vi "PicoScope6000aSettings.vi"(0 "handle in":i16=16384, 1 "Device Info":T3={"PICO_DRIVER_VERSION"="", "PICO_USB_VERSION"="", "PICO_HARDWARE_VERSION"="", "PICO_VARIANT_INFO"="", "PICO_BATCH_AND_SERIAL"="", "PICO_CAL_DATE"="", "PICO_KERNEL_VERSION"="", "PICO_DIGITAL_HARDWARE_VERSION"="", "PICO_ANALOGUE_HARDWARE_VERSION"="", "PICO_FIRMWARE_VERSION_1"="", "PICO_FIRMWARE_VERSION_2"="", "PICO_IPP_VERSION"="", "PICO_DRIVER_PATH"="", "PICO_FIRMWARE_VERSION_3"="", "PICO_FRONT_PANEL_FIRMWARE_VERSION"="", "Number of Channels"=0, "MSO"=TRUE}, 2 "Channels":T2={"Channel A Settings "={"Enabled"=FALSE, "Coupling"=50, "Range"=5, "Analogue Offset"=0.0, "BandWidth"=0}, "Channel B Settings "={"Enabled"=FALSE, "Coupling"=50, "Range"=5, "Analogue Offset"=0.0, "BandWidth"=0}, "Channel C Settings "={"Enabled"=FALSE, "Coupling"=50, "Range"=5, "Analogue Offset"=0.0, "BandWidth"=0}, "Channel D Settings "={"Enabled"=FALSE, "Coupling"=50, "Range"=5, "Analogue Offset"=0.0, "BandWidth"=0}, "Channel E Settings "={"Enabled"=FALSE, "Coupling"=50, "Range"=5, "Analogue Offset"=0.0, "BandWidth"=0}, "Channel F Settings "={"Enabled"=FALSE, "Coupling"=50, "Range"=5, "Analogue Offset"=0.0, "BandWidth"=0}, "Channel G Settings "={"Enabled"=FALSE, "Coupling"=50, "Range"=5, "Analogue Offset"=0.0, "BandWidth"=0}, "Channel H Settings "={"Enabled"=FALSE, "Coupling"=50, "Range"=5, "Analogue Offset"=0.0, "BandWidth"=0}} {"Channel H Settings"."BandWidth" items=["Full"=0, "100kHz"=100000, "20kHz"=200000, "1MHz"=1000000, "20MHz"=20000000, "25MHz"=25000000, "50MHz"=50000000, "200MHz"=200000000, "250MHz"=250000000, "500MHz"=500000000]; "Channel H Settings"."Range" items=["10mV"=0, "20mV"=1, "50mV"=2, "100mV"=3, "200mV"=4, "500mV"=5, "1V"=6, "2V"=7, "5V"=8, "10V"=9, "20V"=10, "50V"=11, "100V"=12, "200V"=13, "x10_Probe_100mV"=32, "x10_Probe_200mV"=33, "x10_Probe_500mV"=34, "x10_Probe_1V"=35, "x10_Probe_2V"=36, "x10_Probe_5V"=37, "x10_Probe_10V"=38, "x10_Probe_20V"=39, "x10_Probe_50V"=40, "x10_Probe_100V"=41, "x10_Probe_200V"=42, "x10_Probe_500V"=43, "CURRENT_CLAMP_60A_2A"=10500, "CURRENT_CLAMP_60A_5A"=10501, "CURRENT_CLAMP_60A_10A"=10502, "CURRENT_CLAMP_60A_20A"=10503, "CURRENT_CLAMP_60A_50A"=10504, "CURRENT_CLAMP_60A_60A"=10505, "CURRENT_CLAMP_60A_V2_0_5A"=10600, "CURRENT_CLAMP_60A_V2_1A"=10601, "CURRENT_CLAMP_60A_V2_2A"=10602, "CURRENT_CLAMP_60A_V2_5A"=10603, "CURRENT_CLAMP_60A_V2_10A"=10604, "CURRENT_CLAMP_60A_V2_20A"=10605, "CURRENT_CLAMP_60A_V2_50A"=10606, "CURRENT_CLAMP_60A_V2_60A"=10607, "RESISTANCE_LEAD_NEG5_TO_20OHM"=7000, "RESISTANCE_LEAD_NEG50_TO_200OHM"=7001, "RESISTANCE_LEAD_NEG500_TO_2KOHM"=7002, "RESISTANCE_LEAD_NEG5K_TO_20KOHM"=7003, "RESISTANCE_LEAD_NEG50K_TO_LEAD_200KOHM"=7004, "RESISTANCE_LEAD_NEG500K_TO_LEAD_2MOHM"=7005, "RESISTANCE_LEAD_DIODE_TEST"=7006, "HT_NEG3_TO_5KV"=8950, "HT_NEG3_TO_10KV"=8951, "HT_NEG5_TO_20KV"=8952, "HT_NEG5_TO_50KV"=8953, "HT_NEG5_TO_100KV"=8954, "HT_NEG3_TO_5KV_INVERTED"=8955, "HT_NEG3_TO_10KV_INVERTED"=8956, "HT_NEG5_TO_20KV_INVERTED"=8957, "HT_NEG5_TO_50KV_INVERTED"=8958, "HT_NEG5_TO_100KV_INVERTED"=8959, "TEMPERATURE_NEG50_TO_150DEGC"=9000, "PRESSURE_SENSOR_-100k-150k_PASCALS"=9100, "PRESSURE_SENSOR_-100k_TO_400k_PASCALS"=9101, "PRESSURE_SENSOR_-200k_TO_800k_PASCALS"=9102, "PRESSURE_SENSOR_-400k_TO_1600k_PASCALS"=9103, "PRESSURE_SENSOR_-400k_TO_3400k_PASCALS"=9104, "PRESSURE_SENSOR_-150k_TO_1350k_PASCALS"=9105]; "Channel H Settings"."Coupling" items=["AC"=0, "DC 1M Ohm"=1, "DC 50 Ohm"=50]; "Channel G Settings"."BandWidth" items=["Full"=0, "100kHz"=100000, "20kHz"=200000, "1MHz"=1000000, "20MHz"=20000000, "25MHz"=25000000, "50MHz"=50000000, "200MHz"=200000000, "250MHz"=250000000, "500MHz"=500000000]; "Channel G Settings"."Range" items=["10mV"=0, "20mV"=1, "50mV"=2, "100mV"=3, "200mV"=4, "500mV"=5, "1V"=6, "2V"=7, "5V"=8, "10V"=9, "20V"=10, "50V"=11, "100V"=12, "200V"=13, "x10_Probe_100mV"=32, "x10_Probe_200mV"=33, "x10_Probe_500mV"=34, "x10_Probe_1V"=35, "x10_Probe_2V"=36, "x10_Probe_5V"=37, "x10_Probe_10V"=38, "x10_Probe_20V"=39, "x10_Probe_50V"=40, "x10_Probe_100V"=41, "x10_Probe_200V"=42, "x10_Probe_500V"=43, "CURRENT_CLAMP_60A_2A"=10500, "CURRENT_CLAMP_60A_5A"=10501, "CURRENT_CLAMP_60A_10A"=10502, "CURRENT_CLAMP_60A_20A"=10503, "CURRENT_CLAMP_60A_50A"=10504, "CURRENT_CLAMP_60A_60A"=10505, "CURRENT_CLAMP_60A_V2_0_5A"=10600, "CURRENT_CLAMP_60A_V2_1A"=10601, "CURRENT_CLAMP_60A_V2_2A"=10602, "CURRENT_CLAMP_60A_V2_5A"=10603, "CURRENT_CLAMP_60A_V2_10A"=10604, "CURRENT_CLAMP_60A_V2_20A"=10605, "CURRENT_CLAMP_60A_V2_50A"=10606, "CURRENT_CLAMP_60A_V2_60A"=10607, "RESISTANCE_LEAD_NEG5_TO_20OHM"=7000, "RESISTANCE_LEAD_NEG50_TO_200OHM"=7001, "RESISTANCE_LEAD_NEG500_TO_2KOHM"=7002, "RESISTANCE_LEAD_NEG5K_TO_20KOHM"=7003, "RESISTANCE_LEAD_NEG50K_TO_LEAD_200KOHM"=7004, "RESISTANCE_LEAD_NEG500K_TO_LEAD_2MOHM"=7005, "RESISTANCE_LEAD_DIODE_TEST"=7006, "HT_NEG3_TO_5KV"=8950, "HT_NEG3_TO_10KV"=8951, "HT_NEG5_TO_20KV"=8952, "HT_NEG5_TO_50KV"=8953, "HT_NEG5_TO_100KV"=8954, "HT_NEG3_TO_5KV_INVERTED"=8955, "HT_NEG3_TO_10KV_INVERTED"=8956, "HT_NEG5_TO_20KV_INVERTED"=8957, "HT_NEG5_TO_50KV_INVERTED"=8958, "HT_NEG5_TO_100KV_INVERTED"=8959, "TEMPERATURE_NEG50_TO_150DEGC"=9000, "PRESSURE_SENSOR_-100k-150k_PASCALS"=9100, "PRESSURE_SENSOR_-100k_TO_400k_PASCALS"=9101, "PRESSURE_SENSOR_-200k_TO_800k_PASCALS"=9102, "PRESSURE_SENSOR_-400k_TO_1600k_PASCALS"=9103, "PRESSURE_SENSOR_-400k_TO_3400k_PASCALS"=9104, "PRESSURE_SENSOR_-150k_TO_1350k_PASCALS"=9105]; "Channel G Settings"."Coupling" items=["AC"=0, "DC 1M Ohm"=1, "DC 50 Ohm"=50]; "Channel F Settings"."BandWidth" items=["Full"=0, "100kHz"=100000, "20kHz"=200000, "1MHz"=1000000, "20MHz"=20000000, "25MHz"=25000000, "50MHz"=50000000, "200MHz"=200000000, "250MHz"=250000000, "500MHz"=500000000]; "Channel F Settings"."Range" items=["10mV"=0, "20mV"=1, "50mV"=2, "100mV"=3, "200mV"=4, "500mV"=5, "1V"=6, "2V"=7, "5V"=8, "10V"=9, "20V"=10, "50V"=11, "100V"=12, "200V"=13, "x10_Probe_100mV"=32, "x10_Probe_200mV"=33, "x10_Probe_500mV"=34, "x10_Probe_1V"=35, "x10_Probe_2V"=36, "x10_Probe_5V"=37, "x10_Probe_10V"=38, "x10_Probe_20V"=39, "x10_Probe_50V"=40, "x10_Probe_100V"=41, "x10_Probe_200V"=42, "x10_Probe_500V"=43, "CURRENT_CLAMP_60A_2A"=10500, "CURRENT_CLAMP_60A_5A"=10501, "CURRENT_CLAMP_60A_10A"=10502, "CURRENT_CLAMP_60A_20A"=10503, "CURRENT_CLAMP_60A_50A"=10504, "CURRENT_CLAMP_60A_60A"=10505, "CURRENT_CLAMP_60A_V2_0_5A"=10600, "CURRENT_CLAMP_60A_V2_1A"=10601, "CURRENT_CLAMP_60A_V2_2A"=10602, "CURRENT_CLAMP_60A_V2_5A"=10603, "CURRENT_CLAMP_60A_V2_10A"=10604, "CURRENT_CLAMP_60A_V2_20A"=10605, "CURRENT_CLAMP_60A_V2_50A"=10606, "CURRENT_CLAMP_60A_V2_60A"=10607, "RESISTANCE_LEAD_NEG5_TO_20OHM"=7000, "RESISTANCE_LEAD_NEG50_TO_200OHM"=7001, "RESISTANCE_LEAD_NEG500_TO_2KOHM"=7002, "RESISTANCE_LEAD_NEG5K_TO_20KOHM"=7003, "RESISTANCE_LEAD_NEG50K_TO_LEAD_200KOHM"=7004, "RESISTANCE_LEAD_NEG500K_TO_LEAD_2MOHM"=7005, "RESISTANCE_LEAD_DIODE_TEST"=7006, "HT_NEG3_TO_5KV"=8950, "HT_NEG3_TO_10KV"=8951, "HT_NEG5_TO_20KV"=8952, "HT_NEG5_TO_50KV"=8953, "HT_NEG5_TO_100KV"=8954, "HT_NEG3_TO_5KV_INVERTED"=8955, "HT_NEG3_TO_10KV_INVERTED"=8956, "HT_NEG5_TO_20KV_INVERTED"=8957, "HT_NEG5_TO_50KV_INVERTED"=8958, "HT_NEG5_TO_100KV_INVERTED"=8959, "TEMPERATURE_NEG50_TO_150DEGC"=9000, "PRESSURE_SENSOR_-100k-150k_PASCALS"=9100, "PRESSURE_SENSOR_-100k_TO_400k_PASCALS"=9101, "PRESSURE_SENSOR_-200k_TO_800k_PASCALS"=9102, "PRESSURE_SENSOR_-400k_TO_1600k_PASCALS"=9103, "PRESSURE_SENSOR_-400k_TO_3400k_PASCALS"=9104, "PRESSURE_SENSOR_-150k_TO_1350k_PASCALS"=9105]; "Channel F Settings"."Coupling" items=["AC"=0, "DC 1M Ohm"=1, "DC 50 Ohm"=50]; "Channel E Settings"."BandWidth" items=["Full"=0, "100kHz"=100000, "20kHz"=200000, "1MHz"=1000000, "20MHz"=20000000, "25MHz"=25000000, "50MHz"=50000000, "200MHz"=200000000, "250MHz"=250000000, "500MHz"=500000000]; "Channel E Settings"."Range" items=["10mV"=0, "20mV"=1, "50mV"=2, "100mV"=3, "200mV"=4, "500mV"=5, "1V"=6, "2V"=7, "5V"=8, "10V"=9, "20V"=10, "50V"=11, "100V"=12, "200V"=13, "x10_Probe_100mV"=32, "x10_Probe_200mV"=33, "x10_Probe_500mV"=34, "x10_Probe_1V"=35, "x10_Probe_2V"=36, "x10_Probe_5V"=37, "x10_Probe_10V"=38, "x10_Probe_20V"=39, "x10_Probe_50V"=40, "x10_Probe_100V"=41, "x10_Probe_200V"=42, "x10_Probe_500V"=43, "CURRENT_CLAMP_60A_2A"=10500, "CURRENT_CLAMP_60A_5A"=10501, "CURRENT_CLAMP_60A_10A"=10502, "CURRENT_CLAMP_60A_20A"=10503, "CURRENT_CLAMP_60A_50A"=10504, "CURRENT_CLAMP_60A_60A"=10505, "CURRENT_CLAMP_60A_V2_0_5A"=10600, "CURRENT_CLAMP_60A_V2_1A"=10601, "CURRENT_CLAMP_60A_V2_2A"=10602, "CURRENT_CLAMP_60A_V2_5A"=10603, "CURRENT_CLAMP_60A_V2_10A"=10604, "CURRENT_CLAMP_60A_V2_20A"=10605, "CURRENT_CLAMP_60A_V2_50A"=10606, "CURRENT_CLAMP_60A_V2_60A"=10607, "RESISTANCE_LEAD_NEG5_TO_20OHM"=7000, "RESISTANCE_LEAD_NEG50_TO_200OHM"=7001, "RESISTANCE_LEAD_NEG500_TO_2KOHM"=7002, "RESISTANCE_LEAD_NEG5K_TO_20KOHM"=7003, "RESISTANCE_LEAD_NEG50K_TO_LEAD_200KOHM"=7004, "RESISTANCE_LEAD_NEG500K_TO_LEAD_2MOHM"=7005, "RESISTANCE_LEAD_DIODE_TEST"=7006, "HT_NEG3_TO_5KV"=8950, "HT_NEG3_TO_10KV"=8951, "HT_NEG5_TO_20KV"=8952, "HT_NEG5_TO_50KV"=8953, "HT_NEG5_TO_100KV"=8954, "HT_NEG3_TO_5KV_INVERTED"=8955, "HT_NEG3_TO_10KV_INVERTED"=8956, "HT_NEG5_TO_20KV_INVERTED"=8957, "HT_NEG5_TO_50KV_INVERTED"=8958, "HT_NEG5_TO_100KV_INVERTED"=8959, "TEMPERATURE_NEG50_TO_150DEGC"=9000, "PRESSURE_SENSOR_-100k-150k_PASCALS"=9100, "PRESSURE_SENSOR_-100k_TO_400k_PASCALS"=9101, "PRESSURE_SENSOR_-200k_TO_800k_PASCALS"=9102, "PRESSURE_SENSOR_-400k_TO_1600k_PASCALS"=9103, "PRESSURE_SENSOR_-400k_TO_3400k_PASCALS"=9104, "PRESSURE_SENSOR_-150k_TO_1350k_PASCALS"=9105]; "Channel E Settings"."Coupling" items=["AC"=0, "DC 1M Ohm"=1, "DC 50 Ohm"=50]; "Channel D Settings"."BandWidth" items=["Full"=0, "100kHz"=100000, "20kHz"=200000, "1MHz"=1000000, "20MHz"=20000000, "25MHz"=25000000, "50MHz"=50000000, "200MHz"=200000000, "250MHz"=250000000, "500MHz"=500000000]; "Channel D Settings"."Range" items=["10mV"=0, "20mV"=1, "50mV"=2, "100mV"=3, "200mV"=4, "500mV"=5, "1V"=6, "2V"=7, "5V"=8, "10V"=9, "20V"=10, "50V"=11, "100V"=12, "200V"=13, "x10_Probe_100mV"=32, "x10_Probe_200mV"=33, "x10_Probe_500mV"=34, "x10_Probe_1V"=35, "x10_Probe_2V"=36, "x10_Probe_5V"=37, "x10_Probe_10V"=38, "x10_Probe_20V"=39, "x10_Probe_50V"=40, "x10_Probe_100V"=41, "x10_Probe_200V"=42, "x10_Probe_500V"=43, "CURRENT_CLAMP_60A_2A"=10500, "CURRENT_CLAMP_60A_5A"=10501, "CURRENT_CLAMP_60A_10A"=10502, "CURRENT_CLAMP_60A_20A"=10503, "CURRENT_CLAMP_60A_50A"=10504, "CURRENT_CLAMP_60A_60A"=10505, "CURRENT_CLAMP_60A_V2_0_5A"=10600, "CURRENT_CLAMP_60A_V2_1A"=10601, "CURRENT_CLAMP_60A_V2_2A"=10602, "CURRENT_CLAMP_60A_V2_5A"=10603, "CURRENT_CLAMP_60A_V2_10A"=10604, "CURRENT_CLAMP_60A_V2_20A"=10605, "CURRENT_CLAMP_60A_V2_50A"=10606, "CURRENT_CLAMP_60A_V2_60A"=10607, "RESISTANCE_LEAD_NEG5_TO_20OHM"=7000, "RESISTANCE_LEAD_NEG50_TO_200OHM"=7001, "RESISTANCE_LEAD_NEG500_TO_2KOHM"=7002, "RESISTANCE_LEAD_NEG5K_TO_20KOHM"=7003, "RESISTANCE_LEAD_NEG50K_TO_LEAD_200KOHM"=7004, "RESISTANCE_LEAD_NEG500K_TO_LEAD_2MOHM"=7005, "RESISTANCE_LEAD_DIODE_TEST"=7006, "HT_NEG3_TO_5KV"=8950, "HT_NEG3_TO_10KV"=8951, "HT_NEG5_TO_20KV"=8952, "HT_NEG5_TO_50KV"=8953, "HT_NEG5_TO_100KV"=8954, "HT_NEG3_TO_5KV_INVERTED"=8955, "HT_NEG3_TO_10KV_INVERTED"=8956, "HT_NEG5_TO_20KV_INVERTED"=8957, "HT_NEG5_TO_50KV_INVERTED"=8958, "HT_NEG5_TO_100KV_INVERTED"=8959, "TEMPERATURE_NEG50_TO_150DEGC"=9000, "PRESSURE_SENSOR_-100k-150k_PASCALS"=9100, "PRESSURE_SENSOR_-100k_TO_400k_PASCALS"=9101, "PRESSURE_SENSOR_-200k_TO_800k_PASCALS"=9102, "PRESSURE_SENSOR_-400k_TO_1600k_PASCALS"=9103, "PRESSURE_SENSOR_-400k_TO_3400k_PASCALS"=9104, "PRESSURE_SENSOR_-150k_TO_1350k_PASCALS"=9105]; "Channel D Settings"."Coupling" items=["AC"=0, "DC 1M Ohm"=1, "DC 50 Ohm"=50]; "Channel C Settings"."BandWidth" items=["Full"=0, "100kHz"=100000, "20kHz"=200000, "1MHz"=1000000, "20MHz"=20000000, "25MHz"=25000000, "50MHz"=50000000, "200MHz"=200000000, "250MHz"=250000000, "500MHz"=500000000]; "Channel C Settings"."Range" items=["10mV"=0, "20mV"=1, "50mV"=2, "100mV"=3, "200mV"=4, "500mV"=5, "1V"=6, "2V"=7, "5V"=8, "10V"=9, "20V"=10, "50V"=11, "100V"=12, "200V"=13, "x10_Probe_100mV"=32, "x10_Probe_200mV"=33, "x10_Probe_500mV"=34, "x10_Probe_1V"=35, "x10_Probe_2V"=36, "x10_Probe_5V"=37, "x10_Probe_10V"=38, "x10_Probe_20V"=39, "x10_Probe_50V"=40, "x10_Probe_100V"=41, "x10_Probe_200V"=42, "x10_Probe_500V"=43, "CURRENT_CLAMP_60A_2A"=10500, "CURRENT_CLAMP_60A_5A"=10501, "CURRENT_CLAMP_60A_10A"=10502, "CURRENT_CLAMP_60A_20A"=10503, "CURRENT_CLAMP_60A_50A"=10504, "CURRENT_CLAMP_60A_60A"=10505, "CURRENT_CLAMP_60A_V2_0_5A"=10600, "CURRENT_CLAMP_60A_V2_1A"=10601, "CURRENT_CLAMP_60A_V2_2A"=10602, "CURRENT_CLAMP_60A_V2_5A"=10603, "CURRENT_CLAMP_60A_V2_10A"=10604, "CURRENT_CLAMP_60A_V2_20A"=10605, "CURRENT_CLAMP_60A_V2_50A"=10606, "CURRENT_CLAMP_60A_V2_60A"=10607, "RESISTANCE_LEAD_NEG5_TO_20OHM"=7000, "RESISTANCE_LEAD_NEG50_TO_200OHM"=7001, "RESISTANCE_LEAD_NEG500_TO_2KOHM"=7002, "RESISTANCE_LEAD_NEG5K_TO_20KOHM"=7003, "RESISTANCE_LEAD_NEG50K_TO_LEAD_200KOHM"=7004, "RESISTANCE_LEAD_NEG500K_TO_LEAD_2MOHM"=7005, "RESISTANCE_LEAD_DIODE_TEST"=7006, "HT_NEG3_TO_5KV"=8950, "HT_NEG3_TO_10KV"=8951, "HT_NEG5_TO_20KV"=8952, "HT_NEG5_TO_50KV"=8953, "HT_NEG5_TO_100KV"=8954, "HT_NEG3_TO_5KV_INVERTED"=8955, "HT_NEG3_TO_10KV_INVERTED"=8956, "HT_NEG5_TO_20KV_INVERTED"=8957, "HT_NEG5_TO_50KV_INVERTED"=8958, "HT_NEG5_TO_100KV_INVERTED"=8959, "TEMPERATURE_NEG50_TO_150DEGC"=9000, "PRESSURE_SENSOR_-100k-150k_PASCALS"=9100, "PRESSURE_SENSOR_-100k_TO_400k_PASCALS"=9101, "PRESSURE_SENSOR_-200k_TO_800k_PASCALS"=9102, "PRESSURE_SENSOR_-400k_TO_1600k_PASCALS"=9103, "PRESSURE_SENSOR_-400k_TO_3400k_PASCALS"=9104, "PRESSURE_SENSOR_-150k_TO_1350k_PASCALS"=9105]; "Channel C Settings"."Coupling" items=["AC"=0, "DC 1M Ohm"=1, "DC 50 Ohm"=50]; "Channel B Settings"."BandWidth" items=["Full"=0, "100kHz"=100000, "20kHz"=200000, "1MHz"=1000000, "20MHz"=20000000, "25MHz"=25000000, "50MHz"=50000000, "200MHz"=200000000, "250MHz"=250000000, "500MHz"=500000000]; "Channel B Settings"."Range" items=["10mV"=0, "20mV"=1, "50mV"=2, "100mV"=3, "200mV"=4, "500mV"=5, "1V"=6, "2V"=7, "5V"=8, "10V"=9, "20V"=10, "50V"=11, "100V"=12, "200V"=13, "x10_Probe_100mV"=32, "x10_Probe_200mV"=33, "x10_Probe_500mV"=34, "x10_Probe_1V"=35, "x10_Probe_2V"=36, "x10_Probe_5V"=37, "x10_Probe_10V"=38, "x10_Probe_20V"=39, "x10_Probe_50V"=40, "x10_Probe_100V"=41, "x10_Probe_200V"=42, "x10_Probe_500V"=43, "CURRENT_CLAMP_60A_2A"=10500, "CURRENT_CLAMP_60A_5A"=10501, "CURRENT_CLAMP_60A_10A"=10502, "CURRENT_CLAMP_60A_20A"=10503, "CURRENT_CLAMP_60A_50A"=10504, "CURRENT_CLAMP_60A_60A"=10505, "CURRENT_CLAMP_60A_V2_0_5A"=10600, "CURRENT_CLAMP_60A_V2_1A"=10601, "CURRENT_CLAMP_60A_V2_2A"=10602, "CURRENT_CLAMP_60A_V2_5A"=10603, "CURRENT_CLAMP_60A_V2_10A"=10604, "CURRENT_CLAMP_60A_V2_20A"=10605, "CURRENT_CLAMP_60A_V2_50A"=10606, "CURRENT_CLAMP_60A_V2_60A"=10607, "RESISTANCE_LEAD_NEG5_TO_20OHM"=7000, "RESISTANCE_LEAD_NEG50_TO_200OHM"=7001, "RESISTANCE_LEAD_NEG500_TO_2KOHM"=7002, "RESISTANCE_LEAD_NEG5K_TO_20KOHM"=7003, "RESISTANCE_LEAD_NEG50K_TO_LEAD_200KOHM"=7004, "RESISTANCE_LEAD_NEG500K_TO_LEAD_2MOHM"=7005, "RESISTANCE_LEAD_DIODE_TEST"=7006, "HT_NEG3_TO_5KV"=8950, "HT_NEG3_TO_10KV"=8951, "HT_NEG5_TO_20KV"=8952, "HT_NEG5_TO_50KV"=8953, "HT_NEG5_TO_100KV"=8954, "HT_NEG3_TO_5KV_INVERTED"=8955, "HT_NEG3_TO_10KV_INVERTED"=8956, "HT_NEG5_TO_20KV_INVERTED"=8957, "HT_NEG5_TO_50KV_INVERTED"=8958, "HT_NEG5_TO_100KV_INVERTED"=8959, "TEMPERATURE_NEG50_TO_150DEGC"=9000, "PRESSURE_SENSOR_-100k-150k_PASCALS"=9100, "PRESSURE_SENSOR_-100k_TO_400k_PASCALS"=9101, "PRESSURE_SENSOR_-200k_TO_800k_PASCALS"=9102, "PRESSURE_SENSOR_-400k_TO_1600k_PASCALS"=9103, "PRESSURE_SENSOR_-400k_TO_3400k_PASCALS"=9104, "PRESSURE_SENSOR_-150k_TO_1350k_PASCALS"=9105]; "Channel B Settings"."Coupling" items=["AC"=0, "DC 1M Ohm"=1, "DC 50 Ohm"=50]; "Channel A Settings"."Range" items=["10mV"=0, "20mV"=1, "50mV"=2, "100mV"=3, "200mV"=4, "500mV"=5, "1V"=6, "2V"=7, "5V"=8, "10V"=9, "20V"=10, "50V"=11, "100V"=12, "200V"=13, "x10_Probe_100mV"=32, "x10_Probe_200mV"=33, "x10_Probe_500mV"=34, "x10_Probe_1V"=35, "x10_Probe_2V"=36, "x10_Probe_5V"=37, "x10_Probe_10V"=38, "x10_Probe_20V"=39, "x10_Probe_50V"=40, "x10_Probe_100V"=41, "x10_Probe_200V"=42, "x10_Probe_500V"=43, "CURRENT_CLAMP_60A_2A"=10500, "CURRENT_CLAMP_60A_5A"=10501, "CURRENT_CLAMP_60A_10A"=10502, "CURRENT_CLAMP_60A_20A"=10503, "CURRENT_CLAMP_60A_50A"=10504, "CURRENT_CLAMP_60A_60A"=10505, "CURRENT_CLAMP_60A_V2_0_5A"=10600, "CURRENT_CLAMP_60A_V2_1A"=10601, "CURRENT_CLAMP_60A_V2_2A"=10602, "CURRENT_CLAMP_60A_V2_5A"=10603, "CURRENT_CLAMP_60A_V2_10A"=10604, "CURRENT_CLAMP_60A_V2_20A"=10605, "CURRENT_CLAMP_60A_V2_50A"=10606, "CURRENT_CLAMP_60A_V2_60A"=10607, "RESISTANCE_LEAD_NEG5_TO_20OHM"=7000, "RESISTANCE_LEAD_NEG50_TO_200OHM"=7001, "RESISTANCE_LEAD_NEG500_TO_2KOHM"=7002, "RESISTANCE_LEAD_NEG5K_TO_20KOHM"=7003, "RESISTANCE_LEAD_NEG50K_TO_LEAD_200KOHM"=7004, "RESISTANCE_LEAD_NEG500K_TO_LEAD_2MOHM"=7005, "RESISTANCE_LEAD_DIODE_TEST"=7006, "HT_NEG3_TO_5KV"=8950, "HT_NEG3_TO_10KV"=8951, "HT_NEG5_TO_20KV"=8952, "HT_NEG5_TO_50KV"=8953, "HT_NEG5_TO_100KV"=8954, "HT_NEG3_TO_5KV_INVERTED"=8955, "HT_NEG3_TO_10KV_INVERTED"=8956, "HT_NEG5_TO_20KV_INVERTED"=8957, "HT_NEG5_TO_50KV_INVERTED"=8958, "HT_NEG5_TO_100KV_INVERTED"=8959, "TEMPERATURE_NEG50_TO_150DEGC"=9000, "PRESSURE_SENSOR_-100k-150k_PASCALS"=9100, "PRESSURE_SENSOR_-100k_TO_400k_PASCALS"=9101, "PRESSURE_SENSOR_-200k_TO_800k_PASCALS"=9102, "PRESSURE_SENSOR_-400k_TO_1600k_PASCALS"=9103, "PRESSURE_SENSOR_-400k_TO_3400k_PASCALS"=9104, "PRESSURE_SENSOR_-150k_TO_1350k_PASCALS"=9105]; "Channel A Settings"."BandWidth" items=["Full"=0, "100kHz"=100000, "20kHz"=200000, "1MHz"=1000000, "20MHz"=20000000, "25MHz"=25000000, "50MHz"=50000000, "200MHz"=200000000, "250MHz"=250000000, "500MHz"=500000000]; "Channel A Settings"."Coupling" items=["AC"=0, "DC 1M Ohm"=1, "DC 50 Ohm"=50]}, 7 "Max ADC value":i16=32512, 11 "error in (no error)":errorcluster, 12 "Trigger Settings":T4={"Trigger Enabled"=FALSE, "Trigger Threshold (Volts/Probe Units)"=0.0, "Trigger Direction"=2, "Trigger Delay (samples)"=0, "Auto Trigger Time (us)"=1000000, "Trigger Source"=0} {"Trigger Source" items=["Channel A"=0, "Channel B"=1, "Channel C"=2, "Channel D"=3, "Channel E"=4, "Channel F"=5, "Channel G"=6, "Channel H"=7, "Trigger AUX"=1001]; "Trigger Direction" items=["Above", "Below", "Rising", "Falling", "Rising or Falling"]; "Trigger Threshold (Volts/Probe Units)" format="%#_6p"}, 14 "Digital Channels":T1={"Port 0 Settings "={"Enabled"=FALSE, "Hysteresis"=3, "Threshold Level (Volts)"=[1.0, 1.0, 1.0, 1.0, 1.0, 1.0, 1.0, 1.0]}, "Port 1 Settings"={"Enabled"=FALSE, "Hysteresis"=3, "Threshold Level (Volts)"=[1.0, 1.0, 1.0, 1.0, 1.0, 1.0, 1.0, 1.0]}} {"Port 1 Settings"."Threshold Level (Volts)" format="%#_4p"; "Port 1 Settings"."Hysteresis" items=["PICO_VERY_HIGH_400MV", "PICO_HIGH_200MV", "PICO_NORMAL_100MV", "PICO_LOW_50MV"]; "Port 0 Settings"."Threshold Level (Volts)" format="%#_4p"; "Port 0 Settings"."Hysteresis" items=["PICO_VERY_HIGH_400MV", "PICO_HIGH_200MV", "PICO_NORMAL_100MV", "PICO_LOW_50MV"]}) -> (3 "Enabled array":i16[](array[numeric])=[1, 0, 0, 0, 0, 0, 0, 0, 0, 0], 4 "handle out":i16=16384, 15 "error out":errorcluster)   [LabVIEW 2010]
doc: "Sets up channels and calls setSimpleTrigger"
uses:
  ps6000a.dll
  PicoScope6000aAnalogChannelSettings.ctl
  PicoScope6000aDigitalChannelSettings.ctl
panel:
  # "D8-D15"
  # "DO-D7"
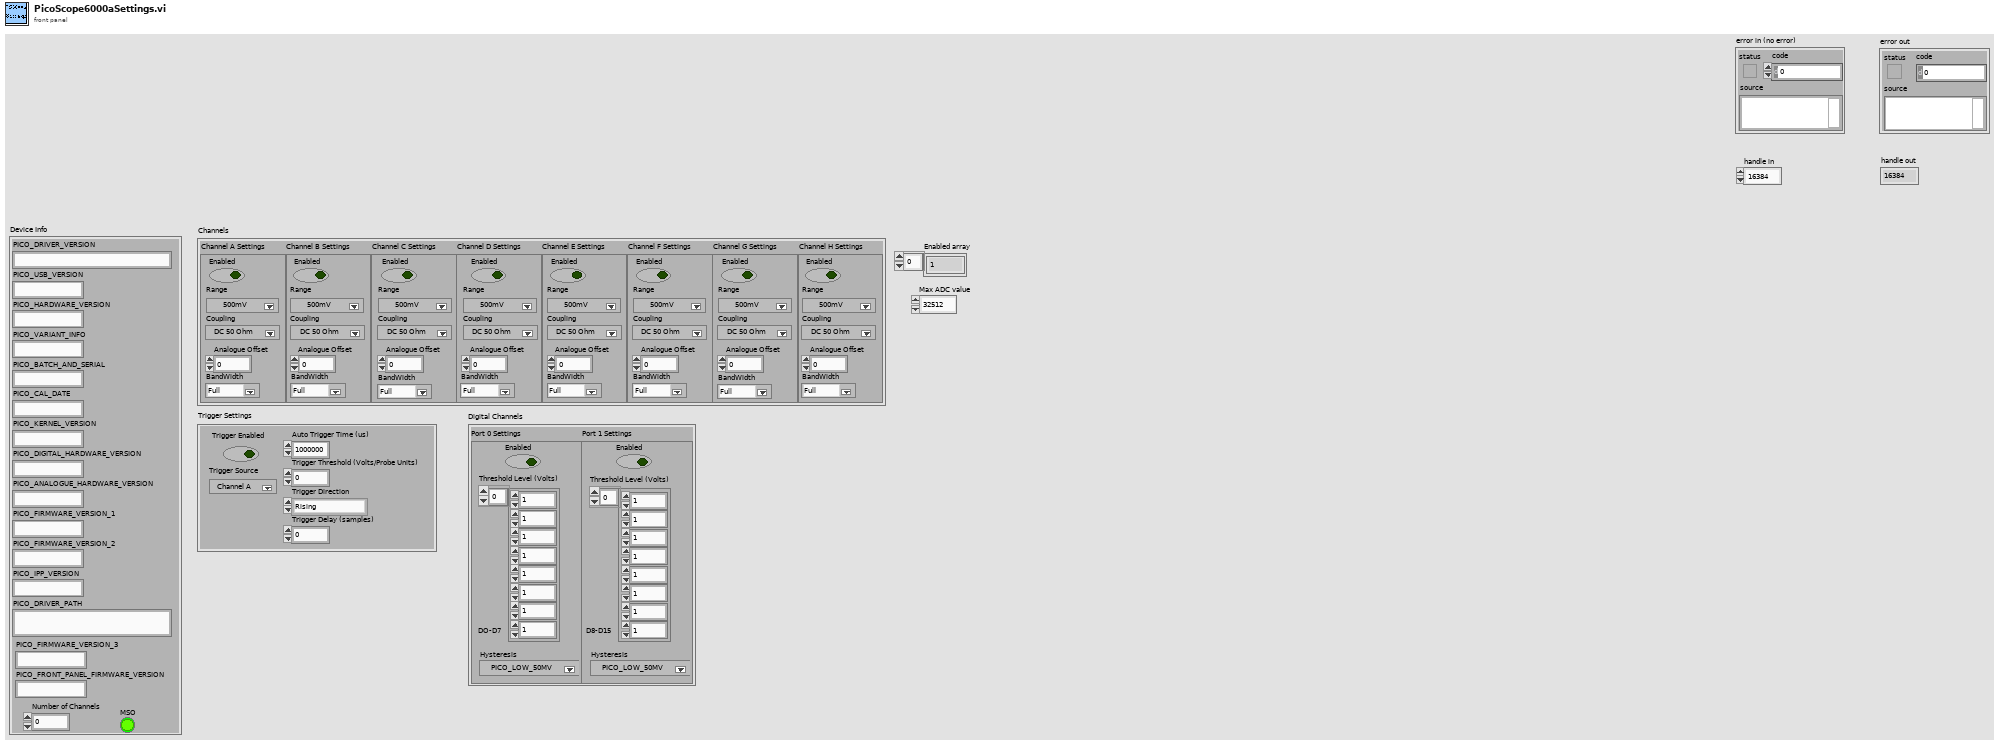
[diagram p1: front panel]
types:
  T1 = typedef "PicoScope6000aDigitalChannelSettings.ctl" = cluster{"Port 0 Settings ":cluster{"Enabled":bool, "Hysteresis":u32, "Threshold Level (Volts)":dbl[]}, "Port 1 Settings":cluster{"Enabled":bool, "Hysteresis":u32, "Threshold Level (Volts)":dbl[]}}
  T2 = typedef "PicoScope6000aAnalogChannelSettings.ctl" = cluster{"Channel A Settings ":cluster{"Enabled":bool, "Coupling":i16, "Range":u32, "Analogue Offset":dbl, "BandWidth":u32}, "Channel B Settings ":cluster{"Enabled":bool, "Coupling":i16, "Range":u32, "Analogue Offset":dbl, "BandWidth":u32}, "Channel C Settings ":cluster{"Enabled":bool, "Coupling":i16, "Range":u32, "Analogue Offset":dbl, "BandWidth":u32}, "Channel D Settings ":cluster{"Enabled":bool, "Coupling":i16, "Range":u32, "Analogue Offset":dbl, "BandWidth":u32}, "Channel E Settings ":cluster{"Enabled":bool, "Coupling":i16, "Range":u32, "Analogue Offset":dbl, "BandWidth":u32}, "Channel F Settings ":cluster{"Enabled":bool, "Coupling":i16, "Range":u32, "Analogue Offset":dbl, "BandWidth":u32}, "Channel G Settings ":cluster{"Enabled":bool, "Coupling":i16, "Range":u32, "Analogue Offset":dbl, "BandWidth":u32}, "Channel H Settings ":cluster{"Enabled":bool, "Coupling":i16, "Range":u32, "Analogue Offset":dbl, "BandWidth":u32}}
  T3 = cluster{"PICO_DRIVER_VERSION":string, "PICO_USB_VERSION":string, "PICO_HARDWARE_VERSION":string, "PICO_VARIANT_INFO":string, "PICO_BATCH_AND_SERIAL":string, "PICO_CAL_DATE":string, "PICO_KERNEL_VERSION":string, "PICO_DIGITAL_HARDWARE_VERSION":string, "PICO_ANALOGUE_HARDWARE_VERSION":string, "PICO_FIRMWARE_VERSION_1":string, "PICO_FIRMWARE_VERSION_2":string, "PICO_IPP_VERSION":string, "PICO_DRIVER_PATH":string, "PICO_FIRMWARE_VERSION_3":string, "PICO_FRONT_PANEL_FIRMWARE_VERSION":string, "Number of Channels":i16, "MSO":bool}
  T4 = cluster{"Trigger Enabled":bool, "Trigger Threshold (Volts/Probe Units)":dbl, "Trigger Direction":u16, "Trigger Delay (samples)":u64, "Auto Trigger Time (us)":u32, "Trigger Source":u32}
  T5 = cluster{"Enabled":bool, "Coupling":i16, "Range":u32, "Analogue Offset":dbl, "BandWidth":u32}
  T6 = cluster{"status":bool, "code":u32, "source":string}
  T7 = cluster{"Enabled":bool, "Hysteresis":u32, "Threshold Level (Volts)":dbl[]}
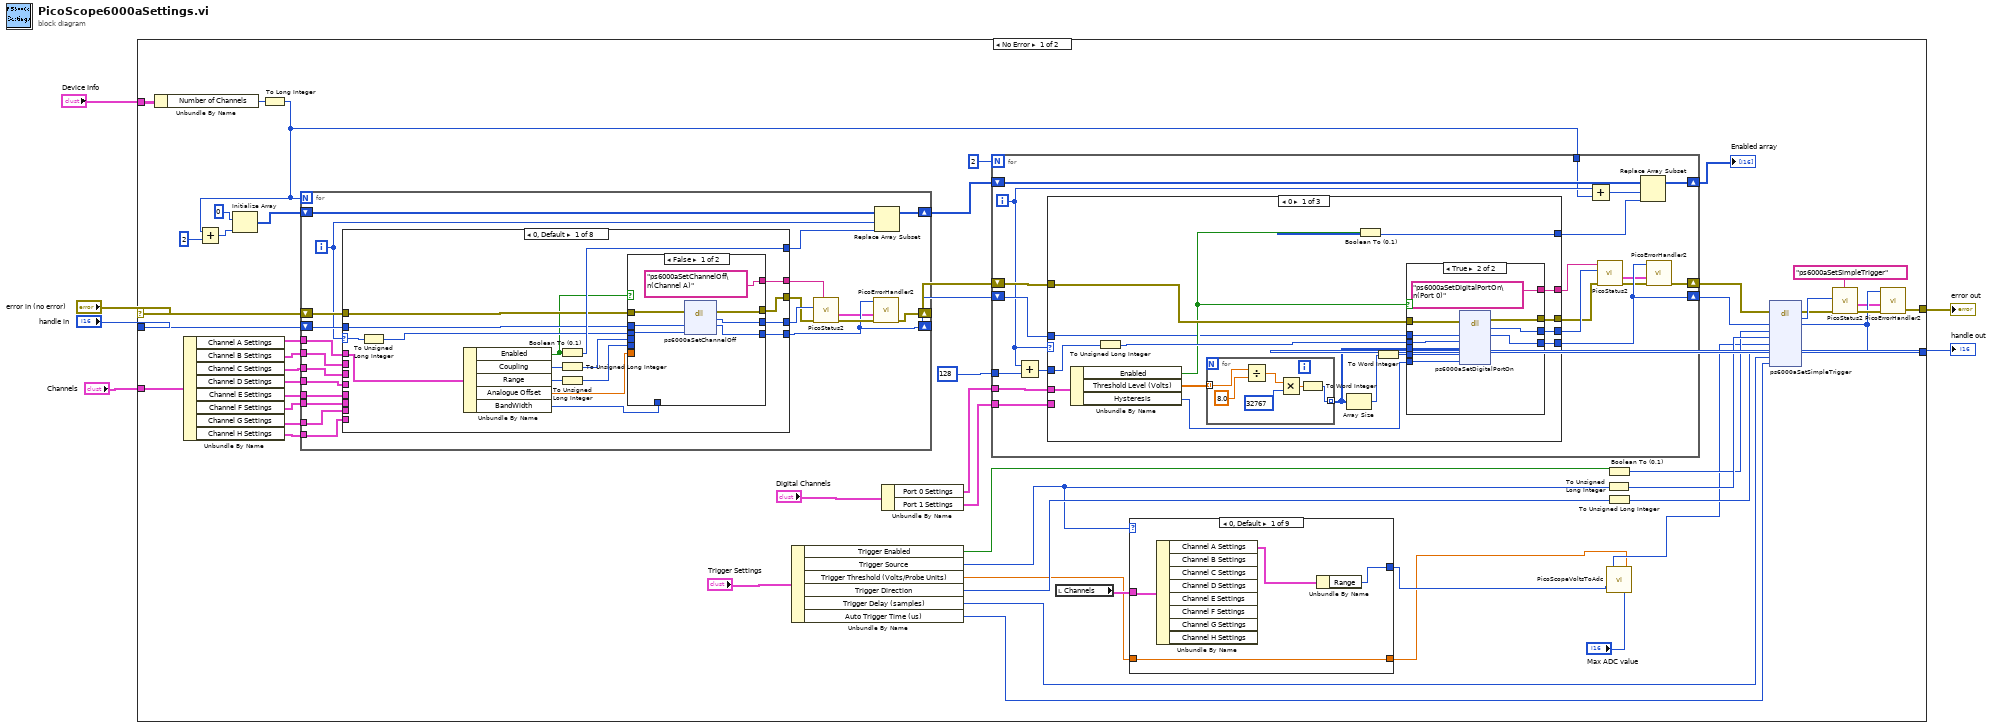
[diagram p0: block diagram]
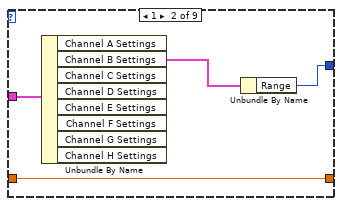
[diagram p2: hidden frame]
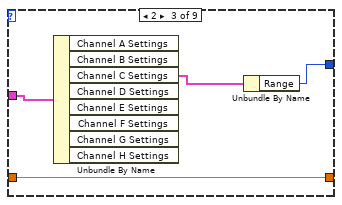
[diagram p3: hidden frame]
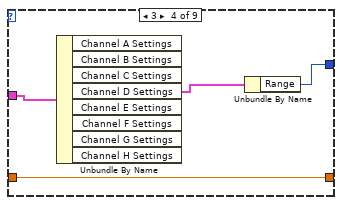
[diagram p4: hidden frame]
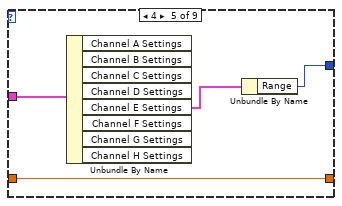
[diagram p5: hidden frame]
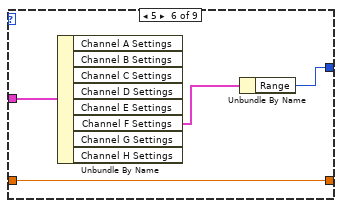
[diagram p6: hidden frame]
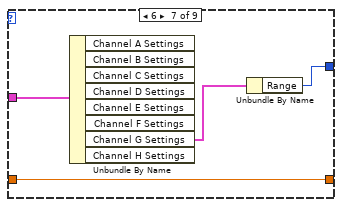
[diagram p7: hidden frame]
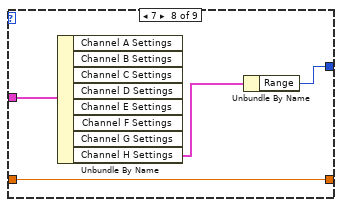
[diagram p8: hidden frame]
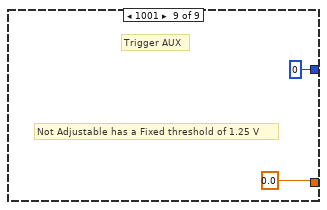
[diagram p9: hidden frame]
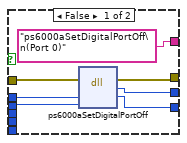
[diagram p10: hidden frame]
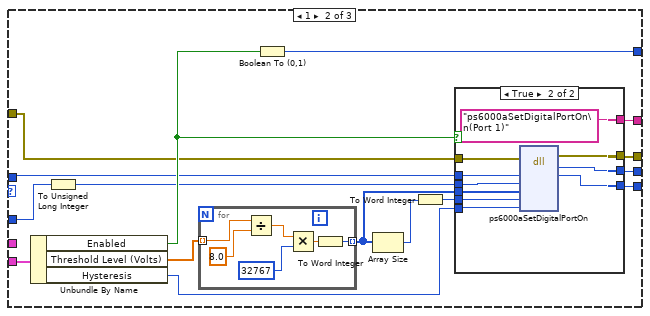
[diagram p11: hidden frame]
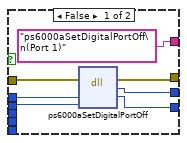
[diagram p12: hidden frame]
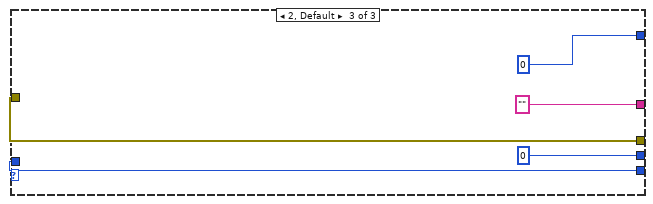
[diagram p13: hidden frame]
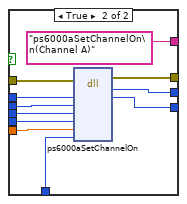
[diagram p14: hidden frame]
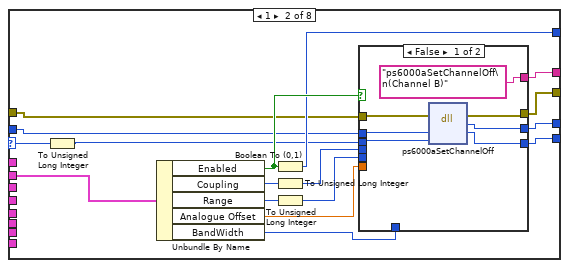
[diagram p15: hidden frame]
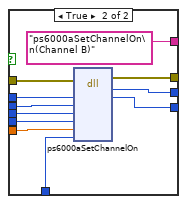
[diagram p16: hidden frame]
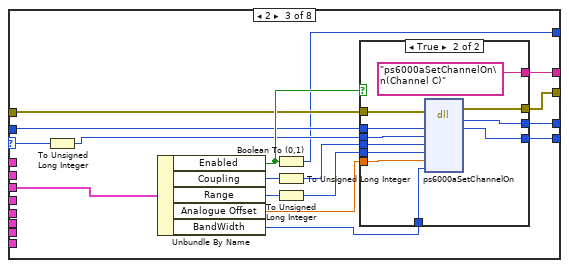
[diagram p17: hidden frame]
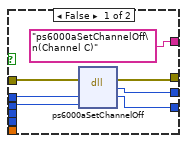
[diagram p18: hidden frame]
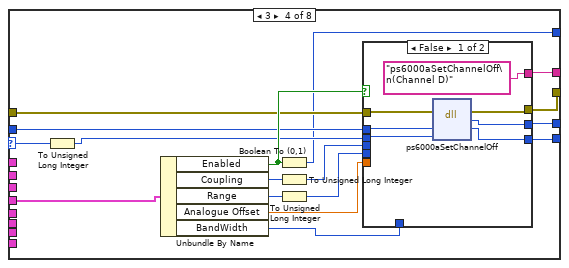
[diagram p19: hidden frame]
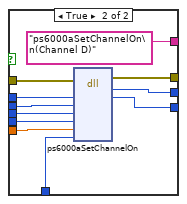
[diagram p20: hidden frame]
diagram:
  n1 = case shown="No Error" "error in (no error)" {
    selector: "error in (no error)" -> [w45 w496]
    tunnel: "handle in" -> [w46 w495]
    tunnel: [w39 w495] -> w6
    tunnel: [w41 w496] -> w5
    tunnel: "Device Info" -> [w42 _]
    tunnel: "Channels" -> [w30 _]
    frame No Error {
      n2 = Unbundle By Name(w42) -> ("Number of Channels"=w9:i16)
      n3 = Unbundle By Name(w30) -> ("Channel A Settings"=w37:T5, "Channel B Settings"=w38:T5, "Channel C Settings"=w36:T5, "Channel D Settings"=w35:T5, "Channel E Settings"=w34:T5, "Channel F Settings"=w31:T5, "Channel G Settings"=w32:T5, "Channel H Settings"=w33:T5)
      n4 = To Long Integer(number=w9) -> (32bit integer=w8:i32)
      n5 = Add(x=w8, y=2) -> (x+y=w11:i32)
      n6 = Initialize Array(i16 0 ("element"), w11) -> (w43:i16[])
      n7 = for {
        N: w8 -> [_]
        shift-right: [w208] -> w25
        shift-left: w45 -> [w213]
        shift-right: [w203] -> w24
        shift-left: w46 -> [w214]
        shift-right: [w209] -> w28
        shift-left: w43 -> [w210]
        tunnel: w38 -> [w202]
        tunnel: w37 -> [w201]
        tunnel: w36 -> [w200]
        tunnel: w35 -> [w199]
        tunnel: w34 -> [w198]
        tunnel: w33 -> [w197]
        tunnel: w32 -> [w196]
        tunnel: w31 -> [w195]
        i -> [w212]
        n8 = case shown="0, Default" w212 {
          selector: w212 -> [w231 w266 w301 w336 w371 w406 w441 w476]
          tunnel: w214 -> [w224 w257 w292 w324 w362 w398 w433 w463]
          tunnel: w213 -> [w226 w258 w293 w329 w363 w397 w432 w464]
          tunnel: [w228 w259 w291 w322 w364 w396 w431 w469] -> w211
          tunnel: [w218 w254 w288 w327 w358 w393 w428 w466] -> w207
          tunnel: [w225 w253 w289 w328 w359 w394 w429 w467] -> w206
          tunnel: [w227 w252 w290 w325 w360 w395 w430 w468] -> w205
          tunnel: [w217 w255 w287 w326 w357 w392 w427 w465] -> w203
          tunnel: w202 -> [_ w251 _ _ _ _ _ _]
          tunnel: w201 -> [w216 _ _ _ _ _ _ _]
          tunnel: w200 -> [_ _ w286 _ _ _ _ _]
          tunnel: w199 -> [_ _ _ w321 _ _ _ _]
          tunnel: w198 -> [_ _ _ _ w356 _ _ _]
          tunnel: w197 -> [_ _ _ _ _ _ _ w461]
          tunnel: w196 -> [_ _ _ _ _ _ w426 _]
          tunnel: w195 -> [_ _ _ _ _ w391 _ _]
          frame 0, Default {
            n9 = To Unsigned Long Integer(number=w231) -> (unsigned 32bit integer=w223:u32)
            n10 = Unbundle By Name(w216) -> ("Enabled"=w219:bool, "Coupling"=w230:i16, "Range"=w229:u32, "Analogue Offset"=w220:dbl, "BandWidth"=w215:u32)
            n11 = Boolean To (0,1)(Boolean=w219) -> (0, 1=w228:i16)
            n12 = To Unsigned Long Integer(number=w230) -> (unsigned 32bit integer=w222:u32)
            n13 = To Unsigned Long Integer(number=w229) -> (unsigned 32bit integer=w221:u32)
            n14 = case shown="False" w219 {
              tunnel: ["ps6000aSetChannelOff\n(Channel A)" ("source") "ps6000aSetChannelOn\n(Channel A)" ("source")] -> w227
              tunnel: w226 -> [w237 w248]
              tunnel: [w236 w247] -> w225
              tunnel: w224 -> [w235 w246]
              tunnel: w223 -> [w234 w245]
              tunnel: w222 -> [_ w244]
              tunnel: w221 -> [_ w243]
              tunnel: w220 -> [_ w242]
              tunnel: [w233 w241] -> w218
              tunnel: [w232 w240] -> w217
              tunnel: w215 -> [_ w239]
              frame False {
                n15 = dll-call lib="ps6000a.dll" fn="ps6000aSetChannelOff" ("ps3000.dll:_ps3000_open_unit@0")(error in=w237, "handle"=w235, "channel"=w234) -> (error out=w236:errorcluster, "PICO_STATUS"=w233:u32, "handle"=w232:i16)  [unwired: 3 in, 1 out]
              }
              frame True {
                n16 = dll-call lib="ps6000a.dll" fn="ps6000aSetChannelOn" ("ps3000.dll:_ps3000_open_unit@0")(error in=w248, "handle"=w246, "channel"=w245, "coupling"=w244, "range"=w243, "analogueOffset"=w242, "bandwidth"=w239) -> (error out=w247:errorcluster, "PICO_STATUS"=w241:u32, "handle"=w240:i16)  [unwired: 7 in, 1 out]
              }
            }
          }
          frame 1 {
            n17 = To Unsigned Long Integer(number=w266) -> (unsigned 32bit integer=w256:u32)
            n18 = Unbundle By Name(w251) -> ("Enabled"=w260:bool, "Coupling"=w265:i16, "Range"=w264:u32, "Analogue Offset"=w261:dbl, "BandWidth"=w250:u32)
            n19 = Boolean To (0,1)(Boolean=w260) -> (0, 1=w259:i16)
            n20 = To Unsigned Long Integer(number=w265) -> (unsigned 32bit integer=w263:u32)
            n21 = To Unsigned Long Integer(number=w264) -> (unsigned 32bit integer=w262:u32)
            n22 = case shown="False" w260 {
              tunnel: ["ps6000aSetChannelOff\n(Channel B)" ("source") "ps6000aSetChannelOn\n(Channel B)" ("source")] -> w252
              tunnel: w258 -> [w272 w283]
              tunnel: [w271 w282] -> w253
              tunnel: w257 -> [w270 w281]
              tunnel: w256 -> [w269 w280]
              tunnel: w263 -> [_ w279]
              tunnel: w262 -> [_ w278]
              tunnel: w261 -> [_ w277]
              tunnel: [w268 w276] -> w254
              tunnel: [w267 w275] -> w255
              tunnel: w250 -> [_ w274]
              frame False {
                n23 = dll-call lib="ps6000a.dll" fn="ps6000aSetChannelOff" ("ps3000.dll:_ps3000_open_unit@0")(error in=w272, "handle"=w270, "channel"=w269) -> (error out=w271:errorcluster, "PICO_STATUS"=w268:u32, "handle"=w267:i16)  [unwired: 3 in, 1 out]
              }
              frame True {
                n24 = dll-call lib="ps6000a.dll" fn="ps6000aSetChannelOn" ("ps3000.dll:_ps3000_open_unit@0")(error in=w283, "handle"=w281, "channel"=w280, "coupling"=w279, "range"=w278, "analogueOffset"=w277, "bandwidth"=w274) -> (error out=w282:errorcluster, "PICO_STATUS"=w276:u32, "handle"=w275:i16)  [unwired: 7 in, 1 out]
              }
            }
          }
          frame 2 {
            n25 = To Unsigned Long Integer(number=w301) -> (unsigned 32bit integer=w294:u32)
            n26 = Unbundle By Name(w286) -> ("Enabled"=w300:bool, "Coupling"=w295:i16, "Range"=w296:u32, "Analogue Offset"=w299:dbl, "BandWidth"=w285:u32)
            n27 = Boolean To (0,1)(Boolean=w300) -> (0, 1=w291:i16)
            n28 = To Unsigned Long Integer(number=w295) -> (unsigned 32bit integer=w297:u32)
            n29 = To Unsigned Long Integer(number=w296) -> (unsigned 32bit integer=w298:u32)
            n30 = case shown="True" w300 {
              tunnel: ["ps6000aSetChannelOff\n(Channel C)" ("source") "ps6000aSetChannelOn\n(Channel C)" ("source")] -> w290
              tunnel: w293 -> [w307 w318]
              tunnel: [w306 w317] -> w289
              tunnel: w292 -> [w305 w316]
              tunnel: w294 -> [w304 w315]
              tunnel: w297 -> [_ w314]
              tunnel: w298 -> [_ w313]
              tunnel: w299 -> [_ w312]
              tunnel: [w303 w311] -> w288
              tunnel: [w302 w310] -> w287
              tunnel: w285 -> [_ w309]
              frame False {
                n31 = dll-call lib="ps6000a.dll" fn="ps6000aSetChannelOff" ("ps3000.dll:_ps3000_open_unit@0")(error in=w307, "handle"=w305, "channel"=w304) -> (error out=w306:errorcluster, "PICO_STATUS"=w303:u32, "handle"=w302:i16)  [unwired: 3 in, 1 out]
              }
              frame True {
                n32 = dll-call lib="ps6000a.dll" fn="ps6000aSetChannelOn" ("ps3000.dll:_ps3000_open_unit@0")(error in=w318, "handle"=w316, "channel"=w315, "coupling"=w314, "range"=w313, "analogueOffset"=w312, "bandwidth"=w309) -> (error out=w317:errorcluster, "PICO_STATUS"=w311:u32, "handle"=w310:i16)  [unwired: 7 in, 1 out]
              }
            }
          }
          frame 3 {
            n33 = To Unsigned Long Integer(number=w336) -> (unsigned 32bit integer=w323:u32)
            n34 = Unbundle By Name(w321) -> ("Enabled"=w330:bool, "Coupling"=w335:i16, "Range"=w334:u32, "Analogue Offset"=w331:dbl, "BandWidth"=w320:u32)
            n35 = Boolean To (0,1)(Boolean=w330) -> (0, 1=w322:i16)
            n36 = To Unsigned Long Integer(number=w335) -> (unsigned 32bit integer=w333:u32)
            n37 = To Unsigned Long Integer(number=w334) -> (unsigned 32bit integer=w332:u32)
            n38 = case shown="False" w330 {
              tunnel: ["ps6000aSetChannelOff\n(Channel D)" ("source") "ps6000aSetChannelOn\n(Channel D)" ("source")] -> w325
              tunnel: w329 -> [w342 w353]
              tunnel: [w341 w352] -> w328
              tunnel: w324 -> [w340 w351]
              tunnel: w323 -> [w339 w350]
              tunnel: w333 -> [_ w349]
              tunnel: w332 -> [_ w348]
              tunnel: w331 -> [_ w347]
              tunnel: [w338 w346] -> w327
              tunnel: [w337 w345] -> w326
              tunnel: w320 -> [_ w344]
              frame False {
                n39 = dll-call lib="ps6000a.dll" fn="ps6000aSetChannelOff" ("ps3000.dll:_ps3000_open_unit@0")(error in=w342, "handle"=w340, "channel"=w339) -> (error out=w341:errorcluster, "PICO_STATUS"=w338:u32, "handle"=w337:i16)  [unwired: 3 in, 1 out]
              }
              frame True {
                n40 = dll-call lib="ps6000a.dll" fn="ps6000aSetChannelOn" ("ps3000.dll:_ps3000_open_unit@0")(error in=w353, "handle"=w351, "channel"=w350, "coupling"=w349, "range"=w348, "analogueOffset"=w347, "bandwidth"=w344) -> (error out=w352:errorcluster, "PICO_STATUS"=w346:u32, "handle"=w345:i16)  [unwired: 7 in, 1 out]
              }
            }
          }
          frame 4 {
            n41 = To Unsigned Long Integer(number=w371) -> (unsigned 32bit integer=w361:u32)
            n42 = Unbundle By Name(w356) -> ("Enabled"=w365:bool, "Coupling"=w370:i16, "Range"=w369:u32, "Analogue Offset"=w366:dbl, "BandWidth"=w355:u32)
            n43 = Boolean To (0,1)(Boolean=w365) -> (0, 1=w364:i16)
            n44 = To Unsigned Long Integer(number=w370) -> (unsigned 32bit integer=w368:u32)
            n45 = To Unsigned Long Integer(number=w369) -> (unsigned 32bit integer=w367:u32)
            n46 = case shown="False" w365 {
              tunnel: ["ps6000aSetChannelOff\n(Channel E)" ("source") "ps6000aSetChannelOn\n(Channel E)" ("source")] -> w360
              tunnel: w363 -> [w377 w388]
              tunnel: [w376 w387] -> w359
              tunnel: w362 -> [w375 w386]
              tunnel: w361 -> [w374 w385]
              tunnel: w368 -> [_ w384]
              tunnel: w367 -> [_ w383]
              tunnel: w366 -> [_ w382]
              tunnel: [w373 w381] -> w358
              tunnel: [w372 w380] -> w357
              tunnel: w355 -> [_ w379]
              frame False {
                n47 = dll-call lib="ps6000a.dll" fn="ps6000aSetChannelOff" ("ps3000.dll:_ps3000_open_unit@0")(error in=w377, "handle"=w375, "channel"=w374) -> (error out=w376:errorcluster, "PICO_STATUS"=w373:u32, "handle"=w372:i16)  [unwired: 3 in, 1 out]
              }
              frame True {
                n48 = dll-call lib="ps6000a.dll" fn="ps6000aSetChannelOn" ("ps3000.dll:_ps3000_open_unit@0")(error in=w388, "handle"=w386, "channel"=w385, "coupling"=w384, "range"=w383, "analogueOffset"=w382, "bandwidth"=w379) -> (error out=w387:errorcluster, "PICO_STATUS"=w381:u32, "handle"=w380:i16)  [unwired: 7 in, 1 out]
              }
            }
          }
          frame 5 {
            n49 = To Unsigned Long Integer(number=w406) -> (unsigned 32bit integer=w399:u32)
            n50 = Unbundle By Name(w391) -> ("Enabled"=w400:bool, "Coupling"=w405:i16, "Range"=w404:u32, "Analogue Offset"=w401:dbl, "BandWidth"=w390:u32)
            n51 = Boolean To (0,1)(Boolean=w400) -> (0, 1=w396:i16)
            n52 = To Unsigned Long Integer(number=w405) -> (unsigned 32bit integer=w403:u32)
            n53 = To Unsigned Long Integer(number=w404) -> (unsigned 32bit integer=w402:u32)
            n54 = case shown="True" w400 {
              tunnel: ["ps6000aSetChannelOff\n(Channel F)" ("source") "ps6000aSetChannelOn\n(Channel F)" ("source")] -> w395
              tunnel: w397 -> [w412 w423]
              tunnel: [w411 w422] -> w394
              tunnel: w398 -> [w410 w421]
              tunnel: w399 -> [w409 w420]
              tunnel: w403 -> [_ w419]
              tunnel: w402 -> [_ w418]
              tunnel: w401 -> [_ w417]
              tunnel: [w408 w416] -> w393
              tunnel: [w407 w415] -> w392
              tunnel: w390 -> [_ w414]
              frame False {
                n55 = dll-call lib="ps6000a.dll" fn="ps6000aSetChannelOff" ("ps3000.dll:_ps3000_open_unit@0")(error in=w412, "handle"=w410, "channel"=w409) -> (error out=w411:errorcluster, "PICO_STATUS"=w408:u32, "handle"=w407:i16)  [unwired: 3 in, 1 out]
              }
              frame True {
                n56 = dll-call lib="ps6000a.dll" fn="ps6000aSetChannelOn" ("ps3000.dll:_ps3000_open_unit@0")(error in=w423, "handle"=w421, "channel"=w420, "coupling"=w419, "range"=w418, "analogueOffset"=w417, "bandwidth"=w414) -> (error out=w422:errorcluster, "PICO_STATUS"=w416:u32, "handle"=w415:i16)  [unwired: 7 in, 1 out]
              }
            }
          }
          frame 6 {
            n57 = To Unsigned Long Integer(number=w441) -> (unsigned 32bit integer=w434:u32)
            n58 = Unbundle By Name(w426) -> ("Enabled"=w435:bool, "Coupling"=w440:i16, "Range"=w439:u32, "Analogue Offset"=w436:dbl, "BandWidth"=w425:u32)
            n59 = Boolean To (0,1)(Boolean=w435) -> (0, 1=w431:i16)
            n60 = To Unsigned Long Integer(number=w440) -> (unsigned 32bit integer=w438:u32)
            n61 = To Unsigned Long Integer(number=w439) -> (unsigned 32bit integer=w437:u32)
            n62 = case shown="True" w435 {
              tunnel: ["ps6000aSetChannelOff\n(Channel G)" ("source") "ps6000aSetChannelOn\n(Channel G)" ("source")] -> w430
              tunnel: w432 -> [w447 w458]
              tunnel: [w446 w457] -> w429
              tunnel: w433 -> [w445 w456]
              tunnel: w434 -> [w444 w455]
              tunnel: w438 -> [_ w454]
              tunnel: w437 -> [_ w453]
              tunnel: w436 -> [_ w452]
              tunnel: [w443 w451] -> w428
              tunnel: [w442 w450] -> w427
              tunnel: w425 -> [_ w449]
              frame False {
                n63 = dll-call lib="ps6000a.dll" fn="ps6000aSetChannelOff" ("ps3000.dll:_ps3000_open_unit@0")(error in=w447, "handle"=w445, "channel"=w444) -> (error out=w446:errorcluster, "PICO_STATUS"=w443:u32, "handle"=w442:i16)  [unwired: 3 in, 1 out]
              }
              frame True {
                n64 = dll-call lib="ps6000a.dll" fn="ps6000aSetChannelOn" ("ps3000.dll:_ps3000_open_unit@0")(error in=w458, "handle"=w456, "channel"=w455, "coupling"=w454, "range"=w453, "analogueOffset"=w452, "bandwidth"=w449) -> (error out=w457:errorcluster, "PICO_STATUS"=w451:u32, "handle"=w450:i16)  [unwired: 7 in, 1 out]
              }
            }
          }
          frame 7 {
            n65 = To Unsigned Long Integer(number=w476) -> (unsigned 32bit integer=w462:u32)
            n66 = Unbundle By Name(w461) -> ("Enabled"=w470:bool, "Coupling"=w475:i16, "Range"=w474:u32, "Analogue Offset"=w471:dbl, "BandWidth"=w460:u32)
            n67 = Boolean To (0,1)(Boolean=w470) -> (0, 1=w469:i16)
            n68 = To Unsigned Long Integer(number=w475) -> (unsigned 32bit integer=w473:u32)
            n69 = To Unsigned Long Integer(number=w474) -> (unsigned 32bit integer=w472:u32)
            n70 = case shown="False" w470 {
              tunnel: ["ps6000aSetChannelOff\n(Channel H)" ("source") "ps6000aSetChannelOn\n(Channel H)" ("source")] -> w468
              tunnel: w464 -> [w482 w493]
              tunnel: [w481 w492] -> w467
              tunnel: w463 -> [w480 w491]
              tunnel: w462 -> [w479 w490]
              tunnel: w473 -> [_ w489]
              tunnel: w472 -> [_ w488]
              tunnel: w471 -> [_ w487]
              tunnel: [w478 w486] -> w466
              tunnel: [w477 w485] -> w465
              tunnel: w460 -> [_ w484]
              frame False {
                n71 = dll-call lib="ps6000a.dll" fn="ps6000aSetChannelOff" ("ps3000.dll:_ps3000_open_unit@0")(error in=w482, "handle"=w480, "channel"=w479) -> (error out=w481:errorcluster, "PICO_STATUS"=w478:u32, "handle"=w477:i16)  [unwired: 3 in, 1 out]
              }
              frame True {
                n72 = dll-call lib="ps6000a.dll" fn="ps6000aSetChannelOn" ("ps3000.dll:_ps3000_open_unit@0")(error in=w493, "handle"=w491, "channel"=w490, "coupling"=w489, "range"=w488, "analogueOffset"=w487, "bandwidth"=w484) -> (error out=w492:errorcluster, "PICO_STATUS"=w486:u32, "handle"=w485:i16)  [unwired: 7 in, 1 out]
              }
            }
          }
        }
        n73 = call "PicoStatus2.vi"("PICO source"=w205, "Error in"=w206, "PICO STATUS"=w207) -> ("error out"=w204:errorcluster, "PICO_STATUS out"=w194:T6)  [unwired: 5 in]
        n74 = call "PicoErrorHandler2.vi"("error in (no error)"=w204, "PICO_STATUS in"=w194, "handle In"=w203) -> ("error out"=w208:errorcluster)  [unwired: 8 in]
        n75 = Replace Array Subset(array=w210, new element=w211, index=w212) -> (w209:i16[])
      }
      n76 = Unbundle By Name("Trigger Settings") -> ("Trigger Enabled"=w51:bool, "Trigger Source"=w15:u32, "Trigger Threshold (Volts/Probe Units)"=w14:dbl, "Trigger Direction"=w54:u16, "Trigger Delay (samples)"=w53:u64, "Auto Trigger Time (us)"=w52:u32)
      n77 = Unbundle By Name("Digital Channels") -> ("Port 0 Settings"=w26:T7, "Port 1 Settings"=w19:T7)
      n78 = for {
        N: 2 -> [_]
        shift-right: [w105] -> w23
        shift-left: w25 -> [w109]
        shift-right: [w101] -> w22
        shift-left: w24 -> [w110]
        shift-right: [w106] -> w29
        shift-left: w28 -> [w107]
        tunnel: w26 -> [w100]
        tunnel: 128 -> [w97]
        tunnel: w19 -> [w95]
        tunnel: w8 -> [w93]
        i -> [w96]
        n79 = Add(x=w96, y=w97) -> (x+y=w98:i32)
        n80 = case shown="0" w96 {
          tunnel: w110 -> [w118 w152 w192]
          tunnel: w109 -> [w124 w154 w193]
          tunnel: [w126 w165 i16 0] -> w108
          tunnel: [w121 w162 u32 0 ("PICO_STATUS")] -> w104
          tunnel: [w123 w163 w193] -> w103
          tunnel: [w125 w164 "" ("source")] -> w102
          tunnel: [w120 w161 w192] -> w101
          tunnel: w100 -> [w115 _ _]
          tunnel: w98 -> [w117 w160 _]
          tunnel: w95 -> [_ w159 _]
          frame 0 {
            n81 = Unbundle By Name(w115) -> ("Enabled"=w119:bool, "Threshold Level (Volts)"=w114:dbl[], "Hysteresis"=w116:u32)
            n82 = To Unsigned Long Integer(number=w117) -> (unsigned 32bit integer=w122:u32)
            n83 = for {
              tunnel: w114 -> [w131] mode=indexing
              tunnel: [w128] -> w111 mode=indexing
              n84 = Divide(x=w131, y=8.0 ("x")) -> (x/y=w132:dbl)
              n85 = Multiply(x=w132, y=i16 32767) -> (x*y=w129:dbl)
              n86 = To Word Integer(number=w129) -> (16bit integer=w128:i16)
            }
            n87 = Array Size(array=w111) -> (size(s)=w112:i32)
            n88 = Boolean To (0,1)(Boolean=w119) -> (0, 1=w126:i16)
            n89 = To Word Integer(number=w112) -> (16bit integer=w113:i16)
            n90 = case shown="True" w119 {
              tunnel: ["ps6000aSetDigitalPortOff\n(Port 0)" ("source") "ps6000aSetDigitalPortOn\n(Port 0)" ("source")] -> w125
              tunnel: w124 -> [w138 w148]
              tunnel: [w137 w147] -> w123
              tunnel: w122 -> [w136 w146]
              tunnel: w111 -> [_ w145]
              tunnel: w113 -> [_ w144]
              tunnel: w116 -> [_ w141]
              tunnel: [w135 w143] -> w121
              tunnel: [w134 w142] -> w120
              tunnel: w118 -> [w133 w140]
              frame False {
                n91 = dll-call lib="ps6000a.dll" fn="ps6000aSetDigitalPortOff" ("ps3000.dll:_ps3000_open_unit@0")(error in=w138, "handle"=w133, "port"=w136) -> (error out=w137:errorcluster, "PICO_STATUS"=w135:u32, "handle"=w134:i16)  [unwired: 3 in, 1 out]
              }
              frame True {
                n92 = dll-call lib="ps6000a.dll" fn="ps6000aSetDigitalPortOn" ("ps3000.dll:_ps3000_open_unit@0")(error in=w148, "handle"=w140, "port"=w146, "logicThresholdLevel"=w145, "logicThresholdLevelLength"=w144, "hysteresis"=w141) -> (error out=w147:errorcluster, "PICO_STATUS"=w143:u32, "handle"=w142:i16)  [unwired: 6 in, 1 out]
              }
            }
          }
          frame 1 {
            n93 = Unbundle By Name(w159) -> ("Enabled"=w155:bool, "Threshold Level (Volts)"=w151:dbl[], "Hysteresis"=w157:u32)
            n94 = To Unsigned Long Integer(number=w160) -> (unsigned 32bit integer=w153:u32)
            n95 = for {
              tunnel: w151 -> [w170] mode=indexing
              tunnel: [w167] -> w150 mode=indexing
              n96 = Divide(x=w170, y=8.0 ("x")) -> (x/y=w171:dbl)
              n97 = Multiply(x=w171, y=i16 32767) -> (x*y=w168:dbl)
              n98 = To Word Integer(number=w168) -> (16bit integer=w167:i16)
            }
            n99 = Boolean To (0,1)(Boolean=w155) -> (0, 1=w165:i16)
            n100 = Array Size(array=w150) -> (size(s)=w158:i32)
            n101 = To Word Integer(number=w158) -> (16bit integer=w156:i16)
            n102 = case shown="True" w155 {
              tunnel: ["ps6000aSetDigitalPortOff\n(Port 1)" ("source") "ps6000aSetDigitalPortOn\n(Port 1)" ("source")] -> w164
              tunnel: w154 -> [w177 w187]
              tunnel: [w176 w186] -> w163
              tunnel: w153 -> [w175 w185]
              tunnel: w150 -> [_ w184]
              tunnel: w156 -> [_ w183]
              tunnel: w157 -> [_ w180]
              tunnel: [w174 w182] -> w162
              tunnel: [w173 w181] -> w161
              tunnel: w152 -> [w172 w179]
              frame False {
                n103 = dll-call lib="ps6000a.dll" fn="ps6000aSetDigitalPortOff" ("ps3000.dll:_ps3000_open_unit@0")(error in=w177, "handle"=w172, "port"=w175) -> (error out=w176:errorcluster, "PICO_STATUS"=w174:u32, "handle"=w173:i16)  [unwired: 3 in, 1 out]
              }
              frame True {
                n104 = dll-call lib="ps6000a.dll" fn="ps6000aSetDigitalPortOn" ("ps3000.dll:_ps3000_open_unit@0")(error in=w187, "handle"=w179, "port"=w185, "logicThresholdLevel"=w184, "logicThresholdLevelLength"=w183, "hysteresis"=w180) -> (error out=w186:errorcluster, "PICO_STATUS"=w182:u32, "handle"=w181:i16)  [unwired: 6 in, 1 out]
              }
            }
          }
          frame 2, Default {
          }
        }
        n105 = Add(x=w96, y=w93) -> (x+y=w94:i32)
        n106 = call "PicoStatus2.vi"("PICO source"=w102, "Error in"=w103, "PICO STATUS"=w104) -> ("error out"=w99:errorcluster, "PICO_STATUS out"=w92:T6)  [unwired: 5 in]
        n107 = Replace Array Subset(array=w107, new element=w108, index=w94) -> (w106:i16[])
        n108 = call "PicoErrorHandler2.vi"("error in (no error)"=w99, "PICO_STATUS in"=w92, "handle In"=w101) -> ("error out"=w105:errorcluster)  [unwired: 8 in]
      }
      "Enabled array" <- w29
      n109 = local read "Channels"() -> (w18:T2)
      n110 = case shown="0, Default" w15 {
        tunnel: [w61 w65 w69 w73 w77 w81 w85 w89 u16 0 ("Range")] -> w13
        tunnel: w18 -> [w60 w64 w68 w72 w76 w80 w84 w88 _]
        tunnel: w14 -> [w58 w62 w66 w70 w74 w78 w82 w86 _]
        tunnel: [w58 w62 w66 w70 w74 w78 w82 w86 0.0 ("Trigger Threshold (Volts/Probe Units)")] -> w12
        frame 0, Default {
          n111 = Unbundle By Name(w60) -> ("Channel A Settings"=w59:T5)  [unwired: 7 out]
          n112 = Unbundle By Name(w59) -> ("Range"=w61:u32)
        }
        frame 1 {
          n113 = Unbundle By Name(w64) -> ("Channel B Settings"=w63:T5)  [unwired: 7 out]
          n114 = Unbundle By Name(w63) -> ("Range"=w65:u32)
        }
        frame 2 {
          n115 = Unbundle By Name(w68) -> ("Channel C Settings"=w67:T5)  [unwired: 7 out]
          n116 = Unbundle By Name(w67) -> ("Range"=w69:u32)
        }
        frame 3 {
          n117 = Unbundle By Name(w72) -> ("Channel D Settings"=w71:T5)  [unwired: 7 out]
          n118 = Unbundle By Name(w71) -> ("Range"=w73:u32)
        }
        frame 4 {
          n119 = Unbundle By Name(w76) -> ("Channel E Settings"=w75:T5)  [unwired: 7 out]
          n120 = Unbundle By Name(w75) -> ("Range"=w77:u32)
        }
        frame 5 {
          n121 = Unbundle By Name(w80) -> ("Channel F Settings"=w79:T5)  [unwired: 7 out]
          n122 = Unbundle By Name(w79) -> ("Range"=w81:u32)
        }
        frame 6 {
          n123 = Unbundle By Name(w84) -> ("Channel G Settings"=w83:T5)  [unwired: 7 out]
          n124 = Unbundle By Name(w83) -> ("Range"=w85:u32)
        }
        frame 7 {
          n125 = Unbundle By Name(w88) -> ("Channel H Settings"=w87:T5)  [unwired: 7 out]
          n126 = Unbundle By Name(w87) -> ("Range"=w89:u32)
        }
        frame 1001 {
          # "Not Adjustable has a Fixed threshold of 1.25 V"
          # "Trigger AUX"
        }
      }
      n127 = To Unsigned Long Integer(number=w15) -> (unsigned 32bit integer=w57:u32)
      n128 = Boolean To (0,1)(Boolean=w51) -> (0, 1=w50:i16)
      n129 = To Unsigned Long Integer(number=w54) -> (unsigned 32bit integer=w56:u32)
      n130 = call "PicoScopeVoltsToAdc.vi"("Max_adc"="Max ADC value", "Units"=w12, "Range Index"=w13) -> ("ADC count"=w16:i16)
      n131 = dll-call lib="ps6000a.dll" fn="ps6000aSetSimpleTrigger" ("ps3000.dll:_ps3000_open_unit@0")(error in=w23, "handle"=w22, "enable"=w50, "source"=w57, "threshold"=w16, "direction"=w56, "delay"=w53, "autoTrigger_us"=w52) -> (error out=w48:errorcluster, "PICO_STATUS"=w49:u32, "handle"=w39:i16)  [unwired: 8 in, 1 out]
      n132 = call "PicoStatus2.vi"("PICO source"="ps6000aSetSimpleTrigger" ("source"), "Error in"=w48, "PICO STATUS"=w49) -> ("error out"=w40:errorcluster, "PICO_STATUS out"=w7:T6)  [unwired: 5 in]
      n133 = call "PicoErrorHandler2.vi"("error in (no error)"=w40, "PICO_STATUS in"=w7, "handle In"=w39) -> ("error out"=w41:errorcluster)  [unwired: 8 in]
    }
    frame Error {
    }
  }
  "error out" <- w5
  "handle out" <- w6
